vi "query ACLR Power Value.vi"(8 "error in (no error)":errorcluster, 10 "Measurement Window Mode":T1=enum."MCACpower", 11 "FSV-40N in":refnum<class "FSV-40N.lvclass">) -> (0 "error out":errorcluster, 2 "Channel Powers":dbl[](array[numeric]), 3 "FSV-40N out":refnum<class "FSV-40N.lvclass">)   [LabVIEW 2023, in "Spectrum Analyzer.lvlib" / "FSV-40N.lvclass"]
uses:
  FSV-40N.lvclass
  TYPE DEFINITION/TYPE Measurement Window Mode.ctl
  FSV-40N.lvclass/FSV-40N.ctl
  Spectrum Analyzer.lvlib
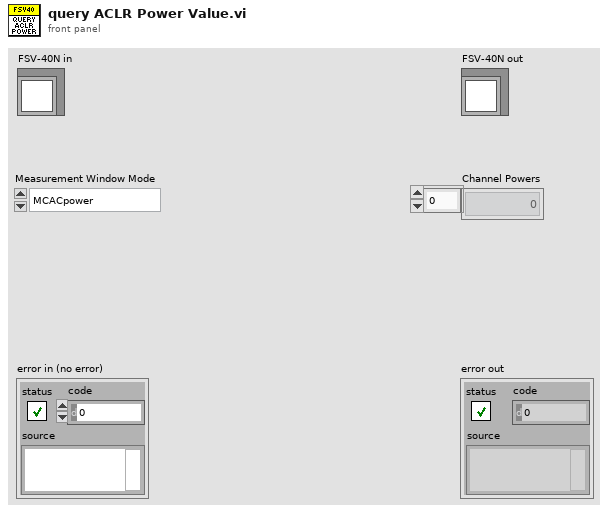
[diagram p1: front panel]
types:
  T1 = typedef "Spectrum Analyzer.lvlib/TYPE Measurement Window Mode.ctl" = enum16{"ACPower", "CPOWer", "MCACpower", "OBANdwidth", "OBWidth", "CN", "CN0"}
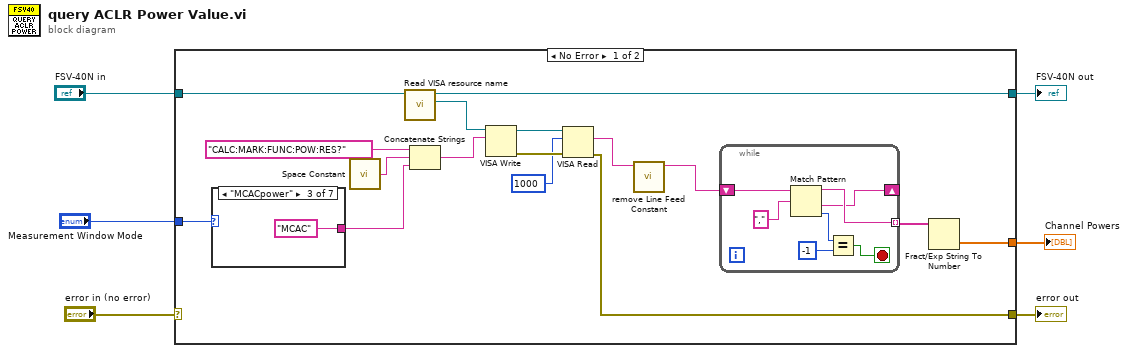
[diagram p0: block diagram]
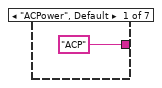
[diagram p2: hidden frame]
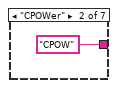
[diagram p3: hidden frame]
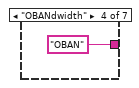
[diagram p4: hidden frame]
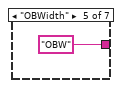
[diagram p5: hidden frame]
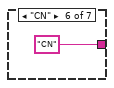
[diagram p6: hidden frame]
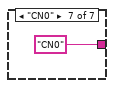
[diagram p7: hidden frame]
diagram:
  n1 = case shown="No Error" "error in (no error)" {
    selector: "error in (no error)" -> [_ w37]
    tunnel: "FSV-40N in" -> [w22 w38]
    tunnel: [w11 w38] -> w4
    tunnel: [w8 w37] -> w3
    tunnel: "Measurement Window Mode" -> [w21 _]
    tunnel: [w7 _] -> w1
    frame No Error {
      n2 = case shown="\"MCACpower\"" w21 {
        tunnel: ["ACP" "CPOW" "MCAC" "OBAN" "OBW" "CN" "CN0"] -> w17
        frame "ACPower", Default {
        }
        frame "CPOWer" {
        }
        frame "MCACpower" {
        }
        frame "OBANdwidth" {
        }
        frame "OBWidth" {
        }
        frame "CN" {
        }
        frame "CN0" {
        }
      }
      n3 = call <vilib>:"Space Constant.vi"() -> ("String"=w18:string)
      n4 = call "Read VISA resource name.vi"("FSV-40N in"=w22) -> ("VISA resource name"=w20:refnum<visa-resource-name>, "FSV-40N out"=w11:refnum<class "FSV-40N.lvclass">)  [unwired: 8 in, 1 out]
      n5 = Concatenate Strings("CALC:MARK:FUNC:POW:RES?" ("string"), w18, w17) -> (w16:string)
      n6 = VISA Write(VISA resource name=w20, write buffer=w16) -> (VISA resource name out=w15:refnum<visa-resource-name>, error out=w14:errorcluster)  [unwired: 1 in, 1 out]
      n7 = VISA Read(VISA resource name=w15, byte count=u32 1000, error in (no error)=w14) -> (read buffer=w12:string, error out=w8:errorcluster)  [unwired: 2 out]
      n8 = call "remove Line Feed Constant.vi"("Input String"=w12) -> ("Line Feed Removed String"=w10:string)  [unwired: 10 in]
      n9 = while {
        shift-right: [w26] -> _
        shift-left: w10 -> [w29]
        tunnel: [w27] -> w9 mode=indexing
        stop <- w25 stop-if-true
        n10 = Match Pattern(string=w29, regular expression=",") -> (before substring=w27:string, after substring=w26:string, offset past match=w24:i32)  [unwired: 1 in, 1 out]
        n11 = Equal?(x=w24, y=-1) -> (x = y?=w25:bool)
      }
      n12 = Fract/Exp String To Number(string=w9) -> (number=w7:dbl[])  [unwired: 3 in, 1 out]
    }
    frame Error {
    }
  }
  "error out" <- w3
  "FSV-40N out" <- w4
  "Channel Powers" <- w1
